vi "GetTestDeviceRbacv3.vi"() -> ()   [LabVIEW 2017]
uses:
  <vilib>/httpClient/LabVIEWHTTPClient.lvlib
panel:
  out "data":cluster{"myInt32":i32, "myBoolean":bool}
  out "error out":errorcluster
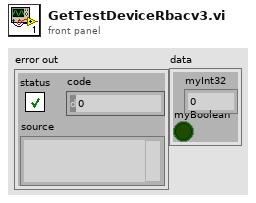
[diagram p1: front panel]
types:
  T1 = typedef "LabVIEWHTTPClient.lvlib/ClientHandle.ctl" = refnum<k1>
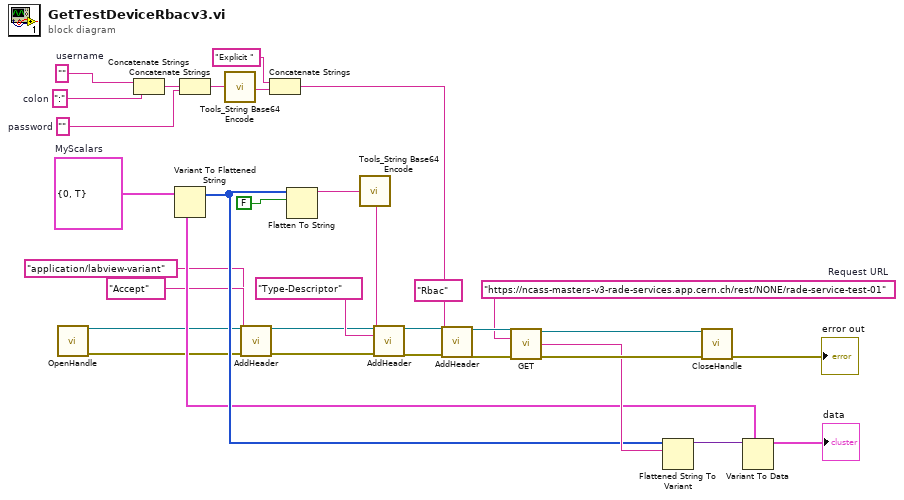
[diagram p0: block diagram]
diagram:
  w13 = "https://ncass-masters-v3-rade-services.app.cern.ch/rest/NONE/rade-service-test-01"  # Request URL
  w26 = ":"  # colon
  w24 = ""  # password
  w27 = ""  # username
  w8 = cluster{"myInt32":i32, "myBoolean":bool} {"myInt32"=0, "myBoolean"=TRUE}  # MyScalars
  n1 = call <vilib>:"OpenHandle.vi"() -> ("client handle out"=w4:T1, "error out"=w3:errorcluster)  [unwired: 14 in]
  n2 = Concatenate Strings(w27, w26) -> (w25:string)
  n3 = Variant To Flattened String(Variant=w8) -> (1:w10:i16[])  [unwired: 1 out]
  n4 = Concatenate Strings(w25, w24) -> (w22:string)
  n5 = call <userlib>:"Tools_String Base64 Encode.vi"("Normal String"=w22) -> ("Base64 String"=w21:string)  [unwired: 1 in]
  n6 = call <vilib>:"AddHeader.vi"("client handle"=w4, "header"="Accept", "value"="application/labview-variant", "error in (no error)"=w3) -> ("client handle out"=w2:T1, "error out"=w1:errorcluster)  [unwired: 10 in]
  n7 = Concatenate Strings("Explicit " ("string"), w21) -> (w20:string)
  n8 = Flatten To String(anything=w10, prepend array or string size? (T)=FALSE) -> (data string=w30:string)  [unwired: 2 in, 2 out]
  n9 = call <userlib>:"Tools_String Base64 Encode.vi"("Normal String"=w30) -> ("Base64 String"=w29:string)  [unwired: 1 in]
  n10 = call <vilib>:"AddHeader.vi"("client handle"=w2, "header"="Type-Descriptor", "value"=w29, "error in (no error)"=w1) -> ("client handle out"=w19:T1, "error out"=w14:errorcluster)  [unwired: 10 in]
  n11 = call <vilib>:"AddHeader.vi"("client handle"=w19, "header"="Rbac", "value"=w20, "error in (no error)"=w14) -> ("client handle out"=w18:T1, "error out"=w15:errorcluster)  [unwired: 10 in]
  n12 = call <vilib>:"GET.vi"("client handle"=w18, "url"=w13, "error in (no error)"=w15) -> ("client handle out"=w17:T1, "body"=w11:string, "error out"=w12:errorcluster)  [unwired: 9 in, 1 out]
  n13 = Flattened String To Variant(6:w11, 7:w10) -> (3:w9:variant)  [unwired: 1 in, 1 out]
  n14 = call <vilib>:"CloseHandle.vi"("client handle"=w17, "error in (no error)"=w12) -> ("error out"=→"error out":errorcluster)  [unwired: 13 in]
  n15 = Variant To Data(type=w8, Variant=w9) -> (data=→"data":cluster{"myInt32":i32, "myBoolean":bool})  [unwired: 1 in, 1 out]
